vi "Main.vi"() -> ()   [LabVIEW 2021]
panel:
  in  "Reset":bool
  in  "New Job":bool
  in  "Welcome":bool
  out "Leds":bool[](array[boolean])
  out "Numéros vérifiés":string[][](table)
  in  "Stop":bool
  in  "Generate":bool
  in  "Check":bool
  out "Numéros générés":string[][](table)
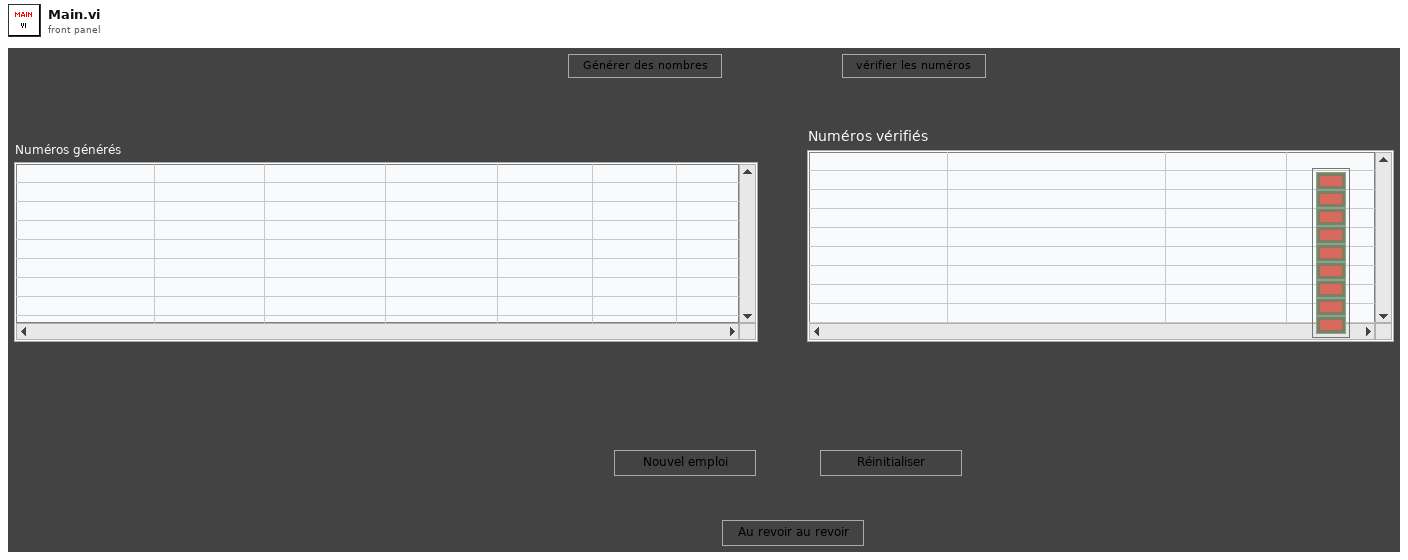
[diagram p1: front panel]
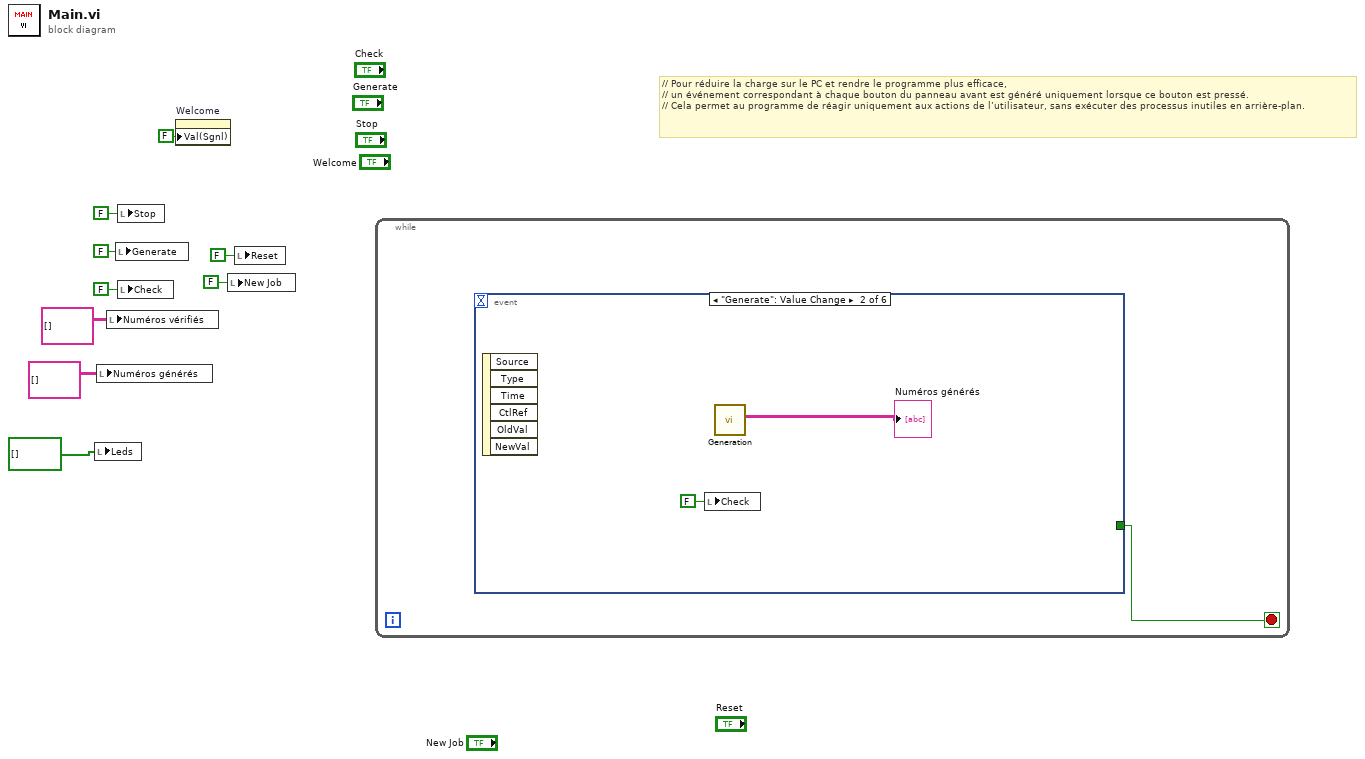
[diagram p0: block diagram]
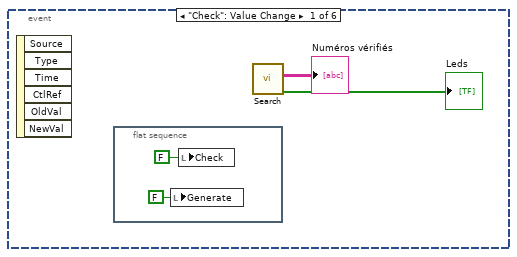
[diagram p2: hidden frame]
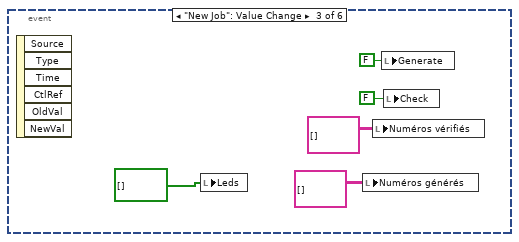
[diagram p3: hidden frame]
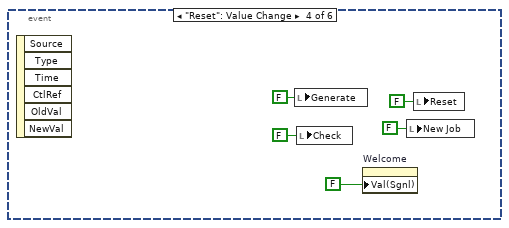
[diagram p4: hidden frame]
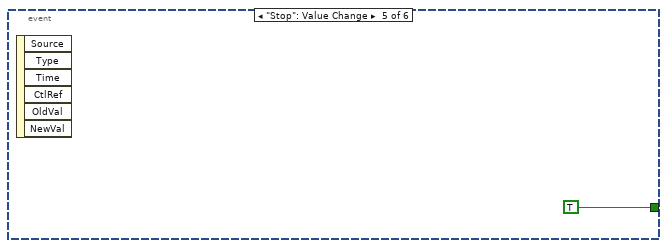
[diagram p5: hidden frame]
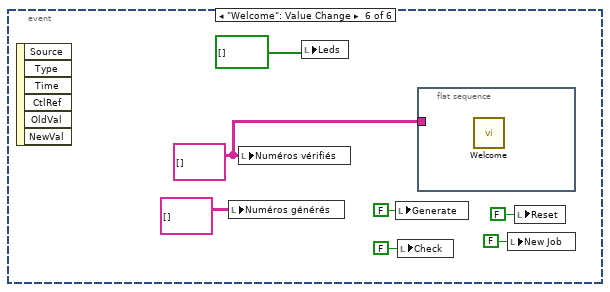
[diagram p6: hidden frame]
diagram:
  # "// Pour réduire la charge sur le PC et rendre le programme plus efficace,\n// un événement correspondant à chaque bouton du panneau avant est généré uniquement lorsque ce bouton est pressé.\n// Cela permet au programme de réagir uniquement aux actions de l’utilisateur, sans exécuter des processus inutiles en arrière-plan."
  n1 = local write "Leds"(bool[] [] ("Leds")) -> ()
  n2 = local write "Numéros générés"(string[][] [] ("Generated Numbers")) -> ()
  n3 = local write "Numéros vérifiés"(string[][] [] ("Numbers checked")) -> ()
  n4 = local write "Generate"(FALSE ("Generate")) -> ()
  n5 = local write "Stop"(FALSE ("Stop")) -> ()
  n6 = local write "Check"(FALSE ("Check")) -> ()
  n7 = property on="Welcome" class="Bool (strict)"("Val(Sgnl)"=FALSE ("Visible")) -> ()  [unwired: 2 in, 2 out]
  n8 = local write "New Job"(FALSE ("New Job")) -> ()
  n9 = local write "Reset"(FALSE ("Reset")) -> ()
  n10 = while {
    stop <- w10 stop-if-true
    n11 = event shown="[1] \"Generate\": Value Change" {
      selector: _ -> [_ _ _ _ _ _]
      dyn-events: _ -> [_ _ _ _ _ _]
      timeout: _ -> [_ _ _ _ _ _]
      tunnel: [_ _ _ _ TRUE _] -> w10
      event "Check": Value Change {
        n12 = event-data() -> ()  [unwired: 1 in, 6 out]
        n13 = flat-sequence {
          frame #0 {
            n14 = local write "Generate"(FALSE ("Generate")) -> ()
            n15 = local write "Check"(FALSE ("Check")) -> ()
          }
        }
        n16 = call "Search.vi"() -> ("data"=→"Numéros vérifiés":string[][], "Leds"=→"Leds":bool[])  [unwired: 9 in]
      }
      event "Generate": Value Change {
        n17 = event-data() -> ()  [unwired: 1 in, 6 out]
        n18 = local write "Check"(FALSE ("Check")) -> ()
        n19 = call "Generation.vi"() -> ("Phone Numbers"=→"Numéros générés":string[][])  [unwired: 11 in]
      }
      event "New Job": Value Change {
        n20 = event-data() -> ()  [unwired: 1 in, 6 out]
        n21 = local write "Leds"(bool[] [] ("Leds")) -> ()
        n22 = local write "Numéros générés"(string[][] [] ("Generated Numbers")) -> ()
        n23 = local write "Numéros vérifiés"(string[][] [] ("Numbers checked")) -> ()
        n24 = local write "Generate"(FALSE ("Generate")) -> ()
        n25 = local write "Check"(FALSE ("Check")) -> ()
      }
      event "Reset": Value Change {
        n26 = event-data() -> ()  [unwired: 1 in, 6 out]
        n27 = local write "Generate"(FALSE ("Generate")) -> ()
        n28 = local write "Check"(FALSE ("Check")) -> ()
        n29 = property on="Welcome" class="Bool (strict)"("Val(Sgnl)"=FALSE ("Visible")) -> ()  [unwired: 2 in, 2 out]
        n30 = local write "New Job"(FALSE ("New Job")) -> ()
        n31 = local write "Reset"(FALSE ("Reset")) -> ()
      }
      event "Stop": Value Change {
        n32 = event-data() -> ()  [unwired: 1 in, 6 out]
      }
      event "Welcome": Value Change {
        w33 = string[][] [] ("Numbers checked")
        n33 = event-data() -> ()  [unwired: 1 in, 6 out]
        n34 = local write "Numéros générés"(string[][] [] ("Generated Numbers")) -> ()
        n35 = local write "Numéros vérifiés"(w33) -> ()
        n36 = local write "Leds"(bool[] [] ("Leds")) -> ()
        n37 = local write "Generate"(FALSE ("Generate")) -> ()
        n38 = local write "Check"(FALSE ("Check")) -> ()
        n39 = flat-sequence {
          tunnel: w33 -> [_]
          frame #0 {
            n40 = call "Welcome.vi"() -> ()  [unwired: 12 in]
          }
        }
        n41 = local write "New Job"(FALSE ("New Job")) -> ()
        n42 = local write "Reset"(FALSE ("Reset")) -> ()
      }
    }
  }
